vi "AdaptToInputs.vi"(3 "Term Types":T1, 4 "XRef":refnum<vi>, 5 "State In":T5) -> (0 "Reply":string[](array[string]), 2 "State Out":T5)   [LabVIEW 2012, in "OpenG Array Sort.xnode"]
uses:
  OpenG Array Sort.xnode
  State.ctl
  <vilib>/XNodeSupport/XNodeTermTypeIDPairs.ctl
  <vilib>/XNodeSupport/XNodeTermTypeIDPair.ctl
  <vilib>/XNodeSupport/XNodeType.ctl
  <vilib>/XNodeSupport/XNodeString.ctl
  <userlib>/_LAVAcr/Scripting Tools/XNode Support/TypeDefs/Array element Tests.ctl
  <userlib>/_LAVAcr/Scripting Tools/XNode Support/Find term type by ID_type.vi
  <userlib>/_LAVAcr/Scripting Tools/XNode Support/XNode Support.lvlib
  <vilib>/XNodeSupport/NI_XNodeSupport.lvlib
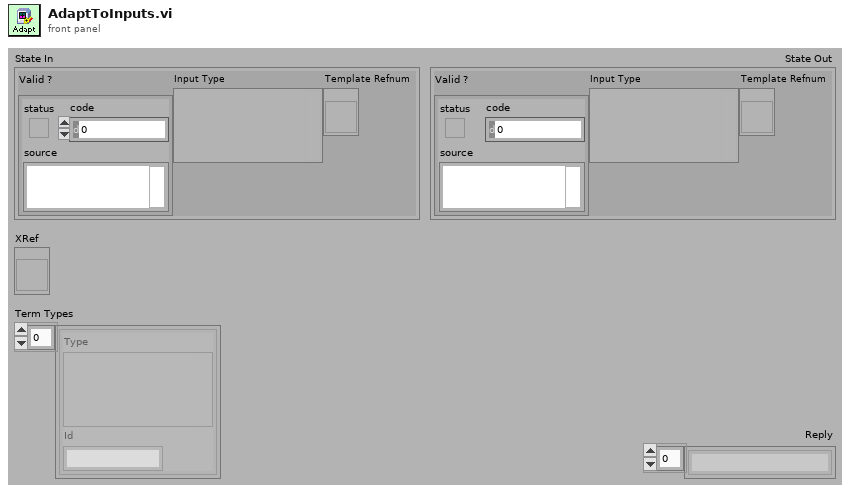
[diagram p1: front panel]
types:
  T1 = typedef "NI_XNodeSupport.lvlib/XNodeTermTypeIDPairs.ctl" = T2[]
  T2 = typedef "NI_XNodeSupport.lvlib/XNodeTermTypeIDPair.ctl" = cluster{"Type":T3, "Id":T4}
  T3 = typedef "NI_XNodeSupport.lvlib/XNodeType.ctl" = variant
  T4 = typedef "NI_XNodeSupport.lvlib/XNodeString.ctl" = string
  T5 = typedef "OpenG Array Sort.xnode/State.ctl" = cluster{"Valid ?":errorcluster, "Input Type":variant, "Template Refnum":refnum<vi>}
  T6 = enum16{"No Check", "At Least n dimensions", "Exactly N Dimensions", "No More Than N Dimensions"}
  T7 = typedef "Scripting Tools.lvlib/XNode Support.lvlib/Array element Tests.ctl" = enum16{"Any Element", "Numeric", "Integer", "Float", "Complex", "Boolean", "String", "Sortable"}
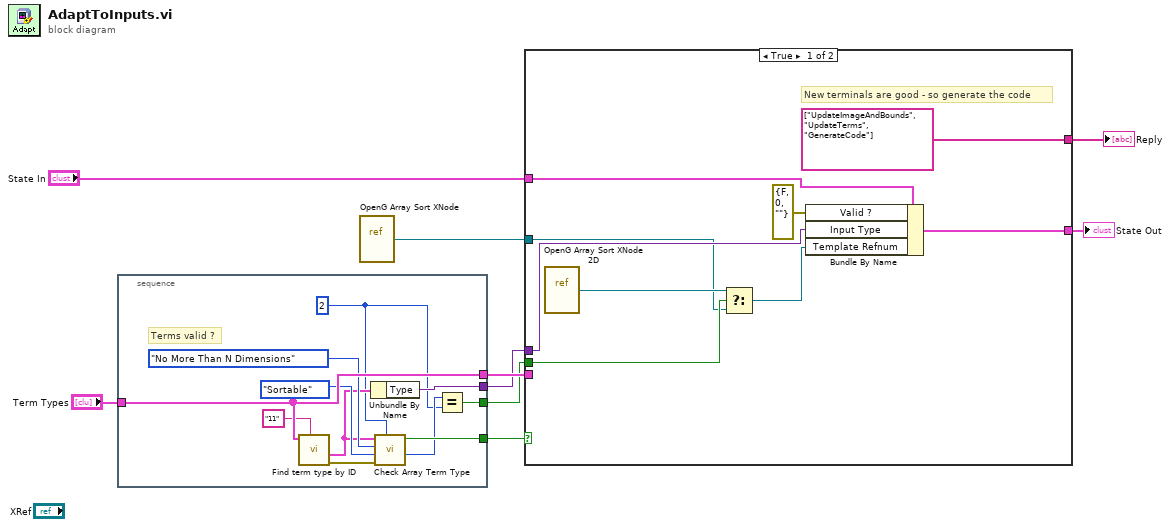
[diagram p0: block diagram]
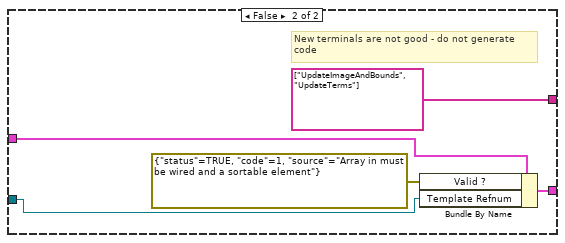
[diagram p2: hidden frame]
diagram:
  n1 = stacked-sequence {
    tunnel: "Term Types" -> [w20]
    tunnel: [w20] -> w7
    tunnel: [w16] -> w8
    tunnel: [w14] -> w3
    tunnel: [w11] -> w2
    frame #0 {
      w12 = 2 ("Dimensions Required")
      # "Terms valid ?"
      n2 = call-poly <userlib>:"Find term type by ID.vi"("Search ID"="11", "Term Types"=w20) -> ("error out"=w10:errorcluster, "Term Type"=w15:T2)  [unwired: 1 in, 7 out]
      n3 = Unbundle By Name(w15) -> ("Type"=w14:T3)
      n4 = call <userlib>:"Check Array Term Type.vi"("Dimensions Required"=w12, "error in (no error)"=w10, "Element Check"=Array_element_Tests."Sortable", "Dimension Check"=T6."No More Than N Dimensions", "Term Type"=w15) -> ("Array Dimensions"=w13:i32, "Is Good ?"=w16:bool)  [unwired: 5 out]
      n5 = Equal?(x=w13, y=w12) -> (x = y?=w11:bool)
    }
  }
  n6 = vi-ref "OpenG Array Sort XNode.vi"() -> (w1:refnum<vi>)
  n7 = case shown="True" w8 {
    tunnel: w7 -> [_ _]
    tunnel: "State In" -> [w29 w34]
    tunnel: [w27 w32] -> w5
    tunnel: [string[] ["UpdateImageAndBounds", "UpdateTerms", "GenerateCode"] ("Reply") string[] ["UpdateImageAndBounds", "UpdateTerms"] ("Reply")] -> w4
    tunnel: w3 -> [w26 _]
    tunnel: w2 -> [w25 _]
    tunnel: w1 -> [w21 w31]
    frame True {
      # "New terminals are good - so generate the code"
      n8 = vi-ref "OpenG Array Sort XNode 2D.vi"() -> (w24:refnum<vi>)
      n9 = Select(t=w24, s=w25, f=w21) -> (s? t:f=w23:refnum<vi>)
      n10 = Bundle By Name(cluster=w29, "Valid ?"=errorcluster {"status"=FALSE, "code"=0, "source"=""}, "Input Type"=w26, "Template Refnum"=w23) -> (w27:T5)
    }
    frame False {
      # "New terminals are not good - do not generate\ncode"
      n11 = Bundle By Name(cluster=w34, "Valid ?"=errorcluster {"status"=TRUE, "code"=1, "source"="Array in must be wired and a sortable element"}, "Template Refnum"=w31) -> (w32:T5)
    }
  }
  "Reply" <- w4
  "State Out" <- w5
